vi "Stop Entry.vi"(6 "Project Store in":refnum<class "Project Store.lvclass">, 7 "Time Entry Store in":refnum<class "Time Entry Store.lvclass">, 8 "error in":errorcluster, 10 "End Time":timestamp, 11 "Active Entry":T1) -> (0 "error out":errorcluster, 2 "Active Entry out":T1, 3 "Stopped Entry":T1, 5 "Time Entry Store out":refnum<class "Time Entry Store.lvclass">)   [LabVIEW 2026]
doc: "Stops the running time entry: sets its End Time and saves it. When Active Entry has an empty ID (nothing is running) nothing is saved and Stopped Entry is Active Entry unchanged. Active Entry out is always a cleared Time Entry (empty IDs, times 0), ready to be stored as the new active entry.\n\nInputs: Active Entry; End Time; Time Entry Store in; Project Store in (optional, supplies the name labels written to the file); error in.\nOutputs: Stopped Entry; Active Entry out; Time Entry Store out; error out.\n\nGenerated by: Claude"
uses:
  Storage/Rows/Time Entry.ctl
  Storage/Time Entry Store/Time Entry Store.lvclass
  Storage/Project Store/Project Store.lvclass
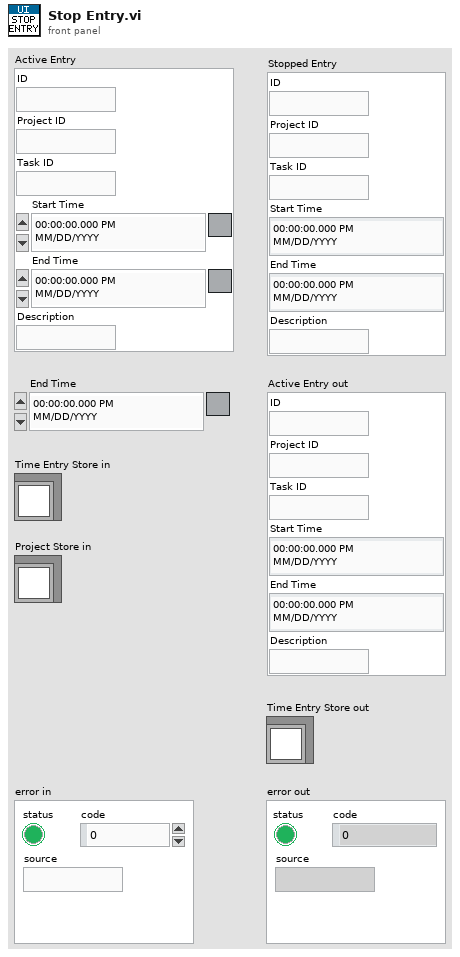
[diagram p1: front panel]
types:
  T1 = typedef "Time Entry.ctl" = cluster{"ID":string, "Project ID":string, "Task ID":string, "Start Time":timestamp, "End Time":timestamp, "Description":string}
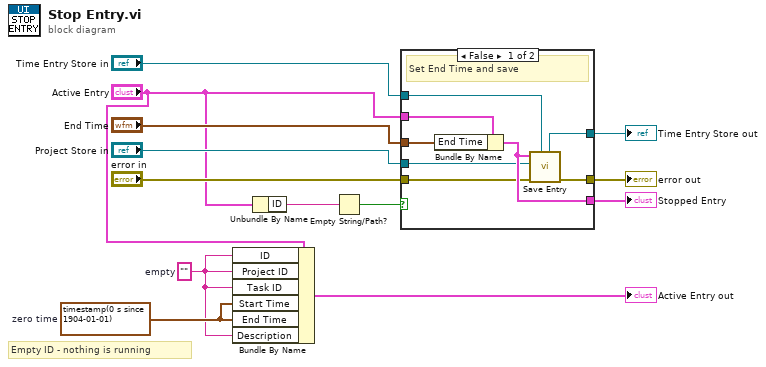
[diagram p0: block diagram]
diagram:
  w11 = timestamp(0 s since 1904-01-01)  # zero time
  w10 = ""  # empty
  # "Empty ID - nothing is running"
  n1 = Bundle By Name(cluster="Active Entry", "ID"=w10, "Project ID"=w10, "Task ID"=w10, "Start Time"=w11, "End Time"=w11, "Description"=w10) -> (→"Active Entry out":T1)
  n2 = Unbundle By Name("Active Entry") -> ("ID"=w12:string)
  n3 = Empty String/Path?(string/path=w12) -> (empty?=w13:bool)
  n4 = case shown="False" w13 {
    tunnel: "Active Entry" -> [w14 w22]
    tunnel: "Time Entry Store in" -> [w15 w23]
    tunnel: "Project Store in" -> [w16 _]
    tunnel: "error in" -> [w17 w24]
    tunnel: "End Time" -> [w18 _]
    tunnel: [w19 w22] -> w6
    tunnel: [w20 w23] -> w8
    tunnel: [w21 w24] -> w9
    frame False {
      # "Set End Time and save"
      n5 = Bundle By Name(cluster=w14, "End Time"=w18) -> (w19:T1)
      n6 = call-dynamic "Save Entry.vi"("Time Entry Store in"=w15, "error in (no error)"=w17, "Project Store"=w16, "Time Entry"=w19) -> ("error out"=w21:errorcluster, "Time Entry Store out"=w20:refnum<class "Time Entry Store.lvclass">)  [unwired: 6 in]
    }
    frame True {
      # "Nothing running - do nothing"
    }
  }
  "Stopped Entry" <- w6
  "Time Entry Store out" <- w8
  "error out" <- w9
